vi "Load Old Configurations.vi"() -> (0 "error out":errorcluster, 2 "Config Matches":bool)   [LabVIEW 2015, in "SystemLink Tag Module tests.lvlib"]
doc: "Test checks whether we are able to deserialize old configurations.\n\nTest should be updated for every configuration version bump."
uses:
  SystemLink Tag Module tests.lvlib
  module/configuration/Data Tag Type.ctl
  <vilib>/NI/Tag Bus/tag/Data Type.ctl
  <vilib>/NI/Tag Bus Module Framework/channel/channel classification.ctl
  module/configuration/SystemLink configuration.lvclass
  module/configuration/SystemLink configuration.lvclass/SystemLink configuration.ctl
  <vilib>/NI/Tag Bus Module Framework/channel/TBM channel.lvclass/TBM channel.ctl
  <vilib>/NI/Tag Bus/tag/tag descriptor.lvclass/tag descriptor.ctl
  module/configuration/Read Prepend Minion ID.vi
  module/configuration/Read Lines.vi
  <vilib>/NI/Tag Bus Module Framework/channel/TBM channel.lvclass
  <vilib>/NI/Tag Bus/tag/tag descriptor.lvclass
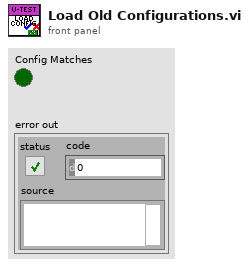
[diagram p1: front panel]
types:
  T1 = typedef "TBM channel.lvclass/channel classification.ctl" = enum16{"input data", "output data", "processing parameter", "processing result"}
  T2 = typedef "tag bus.lvlib/tag descriptor.lvclass/Data Type.ctl" = enum16{"Double", "Single", "I64", "I32", "I16", "I8", "U64", "U32", "U16", "U8", "Boolean", "String", "Array of Double", "Array of Single", "Array of I64", "Array of I32", "Array of I16", "Array of I8", "Array of U64", "Array of U32", "Array of U16", "Array of U8", "Array of Boolean", "Array of String"}
  T3 = typedef "SystemLink configuration.lvclass/Data Tag Type.ctl" = enum16{"Double", "Single", "I32", "I16", "I8", "U64", "U32", "U16", "U8", "Boolean", "String", "Timestamp"}
  T4 = cluster{"Data Tag Type":T3, "channel classification":T1, "data type":T2}
  T5 = typedef "SystemLink configuration.lvclass/Line.ctl" = cluster{"channel":refnum<class "TBM channel.lvclass">, "Data Tag Type":T3}
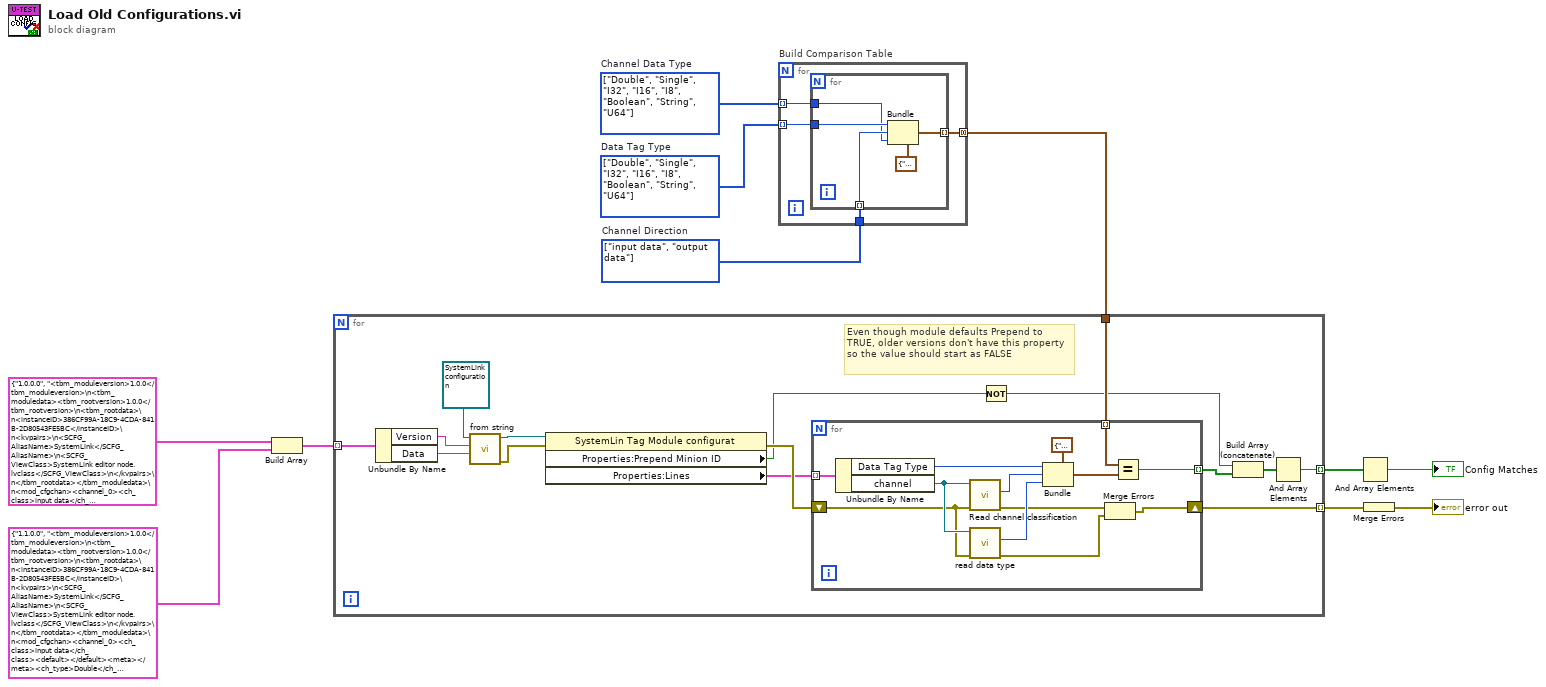
[diagram p0: block diagram]
diagram:
  w8 = T1[] [enum."input data", enum."output data"] items=["input data", "output data", "processing parameter", "processing result"]  # Channel Direction
  w10 = T2[] [enum."Double", enum."Single", enum."I32", enum."I16", enum."I8", enum."Boolean", enum."String", enum."U64"] items=["Double", "Single", "I64", "I32", "I16", "I8", "U64", "U32", "U16", "U8", "Boolean", "String", "Array of Double", "Array of Single", "Array of I64", "Array of I32", "Array of I16", "Array of I8", "Array of U64", "Array of U32", "Array of U16", "Array of U8", "Array of Boolean", "Array of String"]  # Channel Data Type
  w9 = T3[] [enum."Double", enum."Single", enum."I32", enum."I16", enum."I8", enum."Boolean", enum."String", enum."U64"] items=["Double", "Single", "I32", "I16", "I8", "U64", "U32", "U16", "U8", "Boolean", "String", "Timestamp"]  # Data Tag Type
  n1 = Build Array(cluster{"Version":string, "Data":string} {"Version"="1.0.0.0", "Data"="<tbm_moduleversion>1.0.0</tbm_moduleversion>\n<tbm_moduledata><tbm_rootversion>1.0.0</tbm_rootversion>\n<tbm_rootdata>\n<instanceID>386CF99A-18C9-4CDA-841B-2D80543FE5BC</instanceID>\n<kvpairs>\n<SCFG_AliasName>SystemLink</SCFG_AliasName>\n<SCFG_ViewClass>SystemLink editor node.lvclass</SCFG_ViewClass>\n</kvpairs>\n</tbm_rootdata></tbm_moduledata>\n<mod_cfgchan><channel_0><ch_class>input data</ch_class><default></default><meta></meta><ch_type>Double</ch_type><ch_version>1.0.0</ch_version></channel_0><channel_1><ch_class>output data</ch_class><default></default><meta></meta><ch_type>Double</ch_type><ch_version>1.0.0</ch_version></channel_1><channel_2><ch_class>input data</ch_class><default></default><meta></meta><ch_type>Single</ch_type><ch_version>1.0.0</ch_version></channel_2><channel_3><ch_class>output data</ch_class><default></default><meta></meta><ch_type>Single</ch_type><ch_version>1.0.0</ch_version></channel_3><channel_4><ch_class>input data</ch_class><default></default><meta></meta><ch_type>I32</ch_type><ch_version>1.0.0</ch_version></channel_4><channel_5><ch_class>output data</ch_class><default></default><meta></meta><ch_type>I32</ch_type><ch_version>1.0.0</ch_version></channel_5><channel_6><ch_class>input data</ch_class><default></default><meta></meta><ch_type>I16</ch_type><ch_version>1.0.0</ch_version></channel_6><channel_7><ch_class>output data</ch_class><default></default><meta></meta><ch_type>I16</ch_type><ch_version>1.0.0</ch_version></channel_7><channel_8><ch_class>input data</ch_class><default></default><meta></meta><ch_type>I8</ch_type><ch_version>1.0.0</ch_version></channel_8><channel_9><ch_class>output data</ch_class><default></default><meta></meta><ch_type>I8</ch_type><ch_version>1.0.0</ch_version></channel_9><channel_10><ch_class>input data</ch_class><default></default><meta></meta><ch_type>Boolean</ch_type><ch_version>1.0.0</ch_version></channel_10><channel_11><ch_class>output data</ch_class><default></default><meta></meta><ch_type>Boolean</ch_type><ch_version>1.0.0</ch_version></channel_11><channel_12><ch_class>input data</ch_class><default></default><meta></meta><ch_type>String</ch_type><ch_version>1.0.0</ch_version></channel_12><channel_13><ch_class>output data</ch_class><default></default><meta></meta><ch_type>String</ch_type><ch_version>1.0.0</ch_version></channel_13><channel_14><ch_class>input data</ch_class><default></default><meta></meta><ch_type>U64</ch_type><ch_version>1.0.0</ch_version></channel_14><channel_15><ch_class>output data</ch_class><default></default><meta></meta><ch_type>U64</ch_type><ch_version>1.0.0</ch_version></channel_15></mod_cfgchan>"}, cluster{"Version":string, "Data":string} {"Version"="1.1.0.0", "Data"="<tbm_moduleversion>1.0.0</tbm_moduleversion>\n<tbm_moduledata><tbm_rootversion>1.0.0</tbm_rootversion>\n<tbm_rootdata>\n<instanceID>386CF99A-18C9-4CDA-841B-2D80543FE5BC</instanceID>\n<kvpairs>\n<SCFG_AliasName>SystemLink</SCFG_AliasName>\n<SCFG_ViewClass>SystemLink editor node.lvclass</SCFG_ViewClass>\n</kvpairs>\n</tbm_rootdata></tbm_moduledata>\n<mod_cfgchan><channel_0><ch_class>input data</ch_class><default></default><meta></meta><ch_type>Double</ch_type><ch_version>1.0.0</ch_version><ch_datatype>Double</ch_datatype></channel_0><channel_1><ch_class>output data</ch_class><default></default><meta></meta><ch_type>Double</ch_type><ch_version>1.0.0</ch_version><ch_datatype>Double</ch_datatype></channel_1><channel_2><ch_class>input data</ch_class><default></default><meta></meta><ch_type>Single</ch_type><ch_version>1.0.0</ch_version><ch_datatype>Single</ch_datatype></channel_2><channel_3><ch_class>output data</ch_class><default></default><meta></meta><ch_type>Single</ch_type><ch_version>1.0.0</ch_version><ch_datatype>Single</ch_datatype></channel_3><channel_4><ch_class>input data</ch_class><default></default><meta></meta><ch_type>I32</ch_type><ch_version>1.0.0</ch_version><ch_datatype>I32</ch_datatype></channel_4><channel_5><ch_class>output data</ch_class><default></default><meta></meta><ch_type>I32</ch_type><ch_version>1.0.0</ch_version><ch_datatype>I32</ch_datatype></channel_5><channel_6><ch_class>input data</ch_class><default></default><meta></meta><ch_type>I16</ch_type><ch_version>1.0.0</ch_version><ch_datatype>I16</ch_datatype></channel_6><channel_7><ch_class>output data</ch_class><default></default><meta></meta><ch_type>I16</ch_type><ch_version>1.0.0</ch_version><ch_datatype>I16</ch_datatype></channel_7><channel_8><ch_class>input data</ch_class><default></default><meta></meta><ch_type>I8</ch_type><ch_version>1.0.0</ch_version><ch_datatype>I8</ch_datatype></channel_8><channel_9><ch_class>output data</ch_class><default></default><meta></meta><ch_type>I8</ch_type><ch_version>1.0.0</ch_version><ch_datatype>I8</ch_datatype></channel_9><channel_10><ch_class>input data</ch_class><default></default><meta></meta><ch_type>Boolean</ch_type><ch_version>1.0.0</ch_version><ch_datatype>Boolean</ch_datatype></channel_10><channel_11><ch_class>output data</ch_class><default></default><meta></meta><ch_type>Boolean</ch_type><ch_version>1.0.0</ch_version><ch_datatype>Boolean</ch_datatype></channel_11><channel_12><ch_class>input data</ch_class><default></default><meta></meta><ch_type>String</ch_type><ch_version>1.0.0</ch_version><ch_datatype>String</ch_datatype></channel_12><channel_13><ch_class>output data</ch_class><default></default><meta></meta><ch_type>String</ch_type><ch_version>1.0.0</ch_version><ch_datatype>String</ch_datatype></channel_13><channel_14><ch_class>input data</ch_class><default></default><meta></meta><ch_type>U64</ch_type><ch_version>1.0.0</ch_version><ch_datatype>U64</ch_datatype></channel_14><channel_15><ch_class>output data</ch_class><default></default><meta></meta><ch_type>U64</ch_type><ch_version>1.0.0</ch_version><ch_datatype>U64</ch_datatype></channel_15></mod_cfgchan>\n<mod_connection_config><Cluster>\n<Name>Connection Configuration</Name>\n<NumElts>3</NumElts>\n<EW>\n<Name>Connection Type</Name>\n<Choice>AMQP</Choice>\n<Choice>HTTP</Choice>\n<Choice>API Key (SystemLink Cloud)</Choice>\n<Val>0</Val>\n</EW>\n<Cluster>\n<Name>AMQP</Name>\n<NumElts>1</NumElts>\n<String>\n<Name>Configuration ID</Name>\n<Val></Val>\n</String>\n</Cluster>\n<Cluster>\n<Name>HTTP</Name>\n<NumElts>5</NumElts>\n<Boolean>\n<Name>Verify Server?</Name>\n<Val>1</Val>\n</Boolean>\n<String>\n<Name>Server URL</Name>\n<Val></Val>\n</String>\n<String>\n<Name>CA Certificate File</Name>\n<Val></Val>\n</String>\n<Cluster>\n<Name>User Info</Name>\n<NumElts>2</NumElts>\n<String>\n<Name>Username</Name>\n<Val></Val>\n</String>\n<String>\n<Name>Password</Name>\n<Val></Val>\n</String>\n</Cluster>\n<String>\n<Name>API Key</Name>\n<Val></Val>\n</String>\n</Cluster>\n</Cluster>\n</mod_connection_config>"}) -> (w5:cluster{"Version":string, "Data":string}[])
  n2 = for "Build Comparison Table" {
    tunnel: w10 -> [w14] mode=indexing
    tunnel: w9 -> [w13] mode=indexing
    tunnel: w8 -> [w15]
    tunnel: [w12] -> w6 mode=concatenating
    n3 = for {
      tunnel: w15 -> [w18] mode=indexing
      tunnel: w14 -> [w17]
      tunnel: w13 -> [w19]
      tunnel: [w16] -> w12 mode=indexing
      n4 = Bundle(cluster=T4 {"Data Tag Type"=enum."Double", "channel classification"=enum."input data", "data type"=enum."Double"}, "Data Tag Type"=w19, "channel classification"=w18, "data type"=w17) -> (w16:T4)
    }
  }
  n5 = for {
    tunnel: w5 -> [w35] mode=indexing
    tunnel: [w28] -> w7 mode=indexing
    tunnel: w6 -> [w26]
    tunnel: [w25] -> w3 mode=indexing
    # "Even though module defaults Prepend to TRUE, older versions don't have this property so the value should start as FALSE"
    n6 = Unbundle By Name(w35) -> ("Version"=w34:string, "Data"=w33:string)
    n7 = call-dynamic "from string.vi"("data"=w33, "version"=w34, "SystemLin Tag Module configuration in"=refnum<class "SystemLink configuration.lvclass"> refnum ("SystemLin Tag Module configuration")) -> ("error out"=w30:errorcluster, "SystemLin Tag Module configuration out"=w31:refnum<class "SystemLink configuration.lvclass">)  [unwired: 7 in]
    n8 = property class="SystemLin Tag Module configurat"(reference=w31, error in=w30) -> (error out=w29:errorcluster, "Properties:Prepend Minion ID"=w22:bool, "Properties:Lines"=w24:T5[])  [unwired: 1 out]
    n9 = for {
      tunnel: w24 -> [w48] mode=indexing
      shift-right: [w36] -> w28
      shift-left: w29 -> [w46]
      tunnel: w26 -> [w41] mode=indexing
      tunnel: [w39] -> w27 mode=indexing
      n10 = Unbundle By Name(w48) -> ("Data Tag Type"=w44:T3, "channel"=w47:refnum<class "TBM channel.lvclass">)
      n11 = call <vilib>:"Read channel classification.vi"("error in"=w46, "channel in"=w47) -> ("error out"=w38:errorcluster, "channel classification"=w43:T1)  [unwired: 7 in, 1 out]
      n12 = call <vilib>:"read data type.vi"("error in"=w46, "system tag in"=w47) -> ("error out"=w37:errorcluster, "data type"=w42:T2)  [unwired: 7 in, 1 out]
      n13 = Bundle(cluster=T4 {"Data Tag Type"=enum."Double", "channel classification"=enum."input data", "data type"=enum."Double"}, "Data Tag Type"=w44, "channel classification"=w43, "data type"=w42) -> (w40:T4)
      n14 = Merge Errors(w38, w37) -> (w36:errorcluster)
      n15 = Equal?(x=w41, y=w40) -> (x = y?=w39:bool)
    }
    n16 = Not(x=w22) -> (.not. x?=w21:bool)
    n17 = Build Array (concatenate)(w21, w27) -> (w23:bool[])
    n18 = And Array Elements(Boolean array=w23) -> (logical AND=w25:bool)
  }
  n19 = And Array Elements(Boolean array=w3) -> (logical AND=→"Config Matches":bool)
  n20 = Merge Errors(w7) -> (→"error out":errorcluster)
